vi "Read.vi"(8 "error in (no error)":errorcluster, 11 "Boolean in":refnum<class "CTI_GPIO_DigitalIn.lvclass">) -> (0 "error out":errorcluster, 2 "Boolean":bool, 3 "Boolean out":refnum<class "CTI_GPIO_DigitalIn.lvclass">)   [LabVIEW 2021, in "CTI_GPIO_DigitalIn.lvclass"]
doc: "Abstract Data Classes 2.1.1.13\nTim Streeter - TSA\nCopyright (c) 2025, TSA"
uses:
  CTI_GPIO_DigitalIn.lvclass
  CTI_GPIO_DigitalIn.lvclass/CTI_GPIO_DigitalIn.ctl
  <vilib>/CTI/CTI Drivers/CTI/Session/Session.lvclass
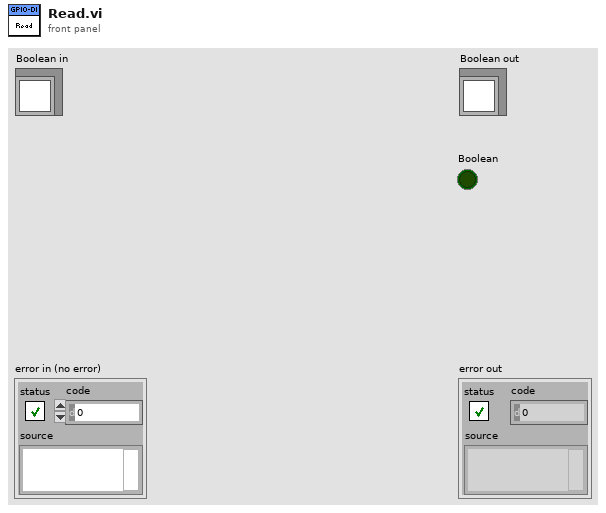
[diagram p1: front panel]
types:
  T1 = typedef "CTI.lvlib/GPIO Number.ctl" = i8
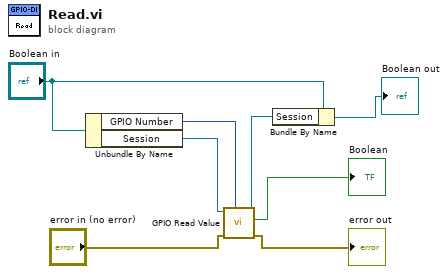
[diagram p0: block diagram]
diagram:
  n1 = Unbundle By Name("Boolean in") -> ("GPIO Number"=w7:T1, "Session"=w8:refnum<class "Session.lvclass">)
  n2 = call <vilib>:"GPIO Read Value.vi"("GPIO #"=w7, "error in (no error)"="error in (no error)", "Session in"=w8) -> ("error out"=→"error out":errorcluster, "Value"=→"Boolean":bool, "Session out"=w3:refnum<class "Session.lvclass">)  [unwired: 6 in]
  n3 = Bundle By Name(cluster="Boolean in", "Session"=w3) -> (→"Boolean out":refnum<class "CTI_GPIO_DigitalIn.lvclass">)
